vi "GetText.vi"(8 "error in":errorcluster, 11 "EthernetIP editor node in":refnum<class "EthernetIP editor node.lvclass">) -> (0 "error out":errorcluster, 1 "additional text":string, 2 "text":string, 3 "EthernetIP editor node out":refnum<class "EthernetIP editor node.lvclass">, 4 "glyph":string)   [LabVIEW 2013, in "EthernetIP editor node.lvclass"]
uses:
  EthernetIP editor node.lvclass
  <vilib>/NI/DCAF/Tag Editor Core/Configuration Editor/PL Framework Configuration Tool.lvlib
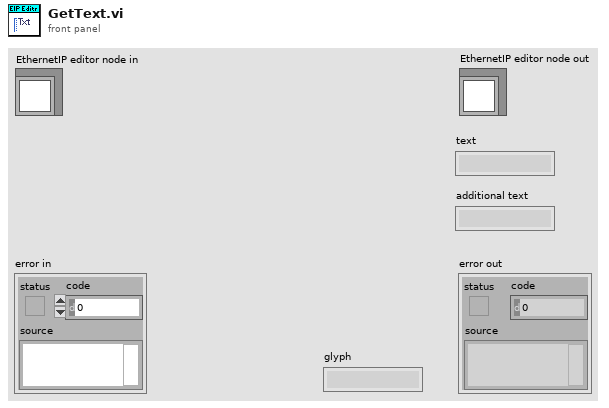
[diagram p1: front panel]
types:
  T1 = typedef "PL Framework Configuration Tool.lvlib/Glyphs Status.ctl" = enum16{"Normal", "Error"}
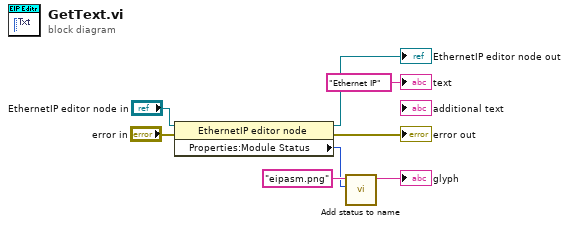
[diagram p0: block diagram]
diagram:
  n1 = property class="EthernetIP editor node"(reference="EthernetIP editor node in", error in="error in") -> (reference out=→"EthernetIP editor node out":refnum<class "EthernetIP editor node.lvclass">, error out=→"error out":errorcluster, "Properties:Module Status"=w7:T1)
  n2 = call <vilib>:"Add status to name.vi"("Status"=w7, "Name"="eipasm.png" ("glyph")) -> ("Name with status"=→"glyph":string)  [unwired: 9 in]
  "text" <- "Ethernet IP" ("text")
